vi "calculate_strain_from_array_normalized2__36f923f621.vi"(7 "real strain":dbl[](array[numeric]), 9 "Gap":dbl, 10 "voltage to displacement contant":dbl) -> (2 "real strain (-)":dbl[](array[numeric]))   [LabVIEW 2023]
panel:
  in  "Numeric":dbl
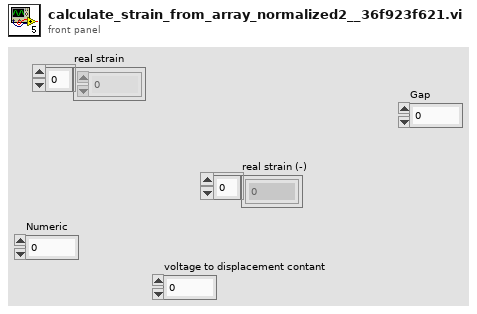
[diagram p1: front panel]
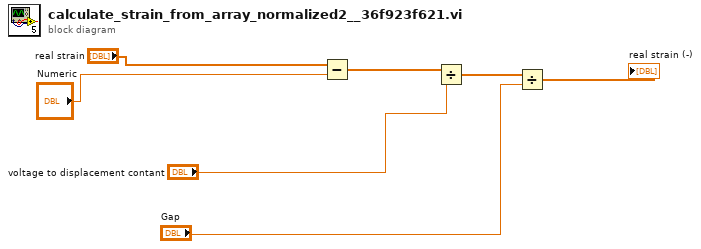
[diagram p0: block diagram]
diagram:
  n1 = Subtract(x="real strain", y="Numeric") -> (x-y=w5:dbl[])
  n2 = Divide(x=w5, y="voltage to displacement contant") -> (x/y=w6:dbl[])
  n3 = Divide(x=w6, y="Gap") -> (x/y=→"real strain (-)":dbl[])
